vi "query Uplink Channel Number.vi"(8 "error in (no error)":errorcluster, 9 "UL Channel Arguments":T2, 11 "LTE in":refnum<class "LTE.lvclass">) -> (0 "error out":errorcluster, 2 "UL Channel Info":T1, 3 "LTE out":refnum<class "LTE.lvclass">)   [LabVIEW 2023, in "ANRITSU Call Box.lvlib" / "LTE.lvclass"]
uses:
  LTE.lvclass
  LTE.lvclass/LTE.ctl
  ANRITSU Call Box.lvlib
  Type Definition/LTE Uplink Channel Number Info.ctl
  Type Definition/LTE Uplink Channel Number Target.ctl
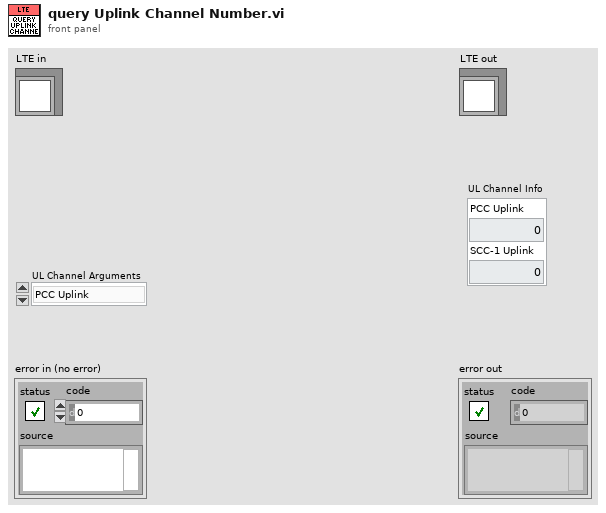
[diagram p1: front panel]
types:
  T1 = typedef "ANRITSU Call Box.lvlib/LTE Uplink Channel Number Info.ctl" = cluster{"PCC Uplink":i32, "SCC-1 Uplink":i32}
  T2 = typedef "ANRITSU Call Box.lvlib/LTE Uplink Channel Number Target.ctl" = enum16{"PCC Uplink", "SCC-1 Uplink", "All"}
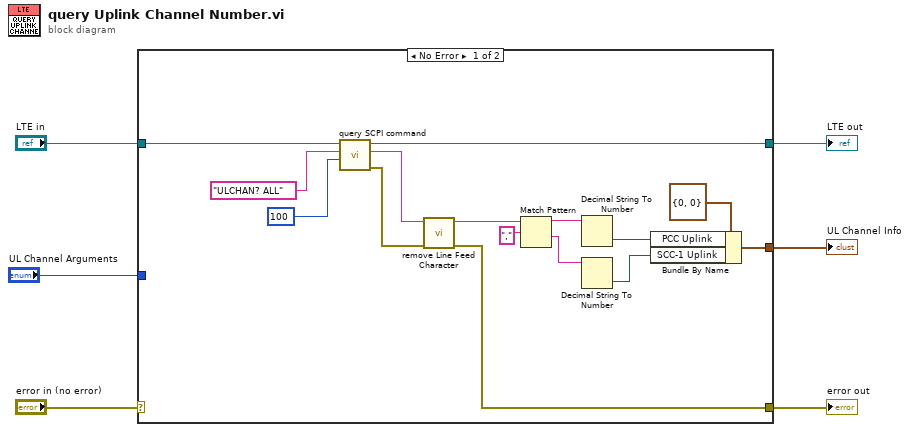
[diagram p0: block diagram]
diagram:
  n1 = case shown="No Error" "error in (no error)" {
    selector: "error in (no error)" -> [_ w23]
    tunnel: [w7 w23] -> w5
    tunnel: [w20 w22] -> w3
    tunnel: "LTE in" -> [w21 w22]
    tunnel: "UL Channel Arguments" -> [_ _]
    tunnel: [w8 _] -> w1
    frame No Error {
      n2 = call "query SCPI command.vi"("Read Buffer Length"=u32 100, "SCPI Command"="ULCHAN? ALL" ("string"), "LTE in"=w21) -> ("error out"=w16:errorcluster, "Read Buffer String"=w17:string, "LTE out"=w20:refnum<class "LTE.lvclass">)  [unwired: 6 in]
      n3 = call "remove Line Feed Character.vi"("error in"=w16, "Query String"=w17) -> ("error out"=w7:errorcluster, "Line Feed Removed String"=w12:string)  [unwired: 8 in]
      n4 = Match Pattern(string=w12, regular expression=",") -> (before substring=w14:string, after substring=w13:string)  [unwired: 1 in, 2 out]
      n5 = Decimal String To Number(string=w14) -> (number=w10:i32)  [unwired: 2 in, 1 out]
      n6 = Decimal String To Number(string=w13) -> (number=w9:i32)  [unwired: 2 in, 1 out]
      n7 = Bundle By Name(cluster=T1 {"PCC Uplink"=0, "SCC-1 Uplink"=0} ("UL Channel Info 2"), "PCC Uplink"=w10, "SCC-1 Uplink"=w9) -> (w8:T1)
    }
    frame Error {
    }
  }
  "error out" <- w5
  "LTE out" <- w3
  "UL Channel Info" <- w1
